vi "JudgeVoltage.vi"(9 "High_mV":i32, 10 "Low_mV":i32, 11 "Voltage_mV":i32) -> (2 "InputValid":bool, 3 "Result":u16)   [LabVIEW 2026]
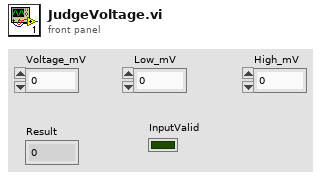
[diagram p1: front panel]
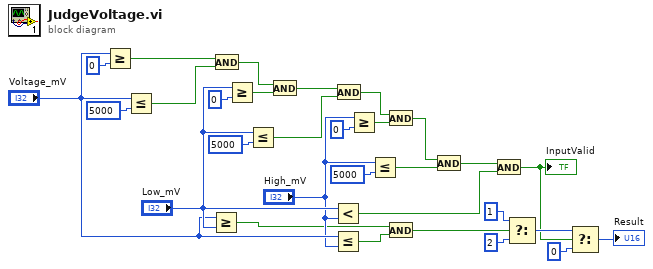
[diagram p0: block diagram]
diagram:
  n1 = Greater Or Equal?(x="Voltage_mV", y=0) -> (x >= y?=w24:bool)
  n2 = Less Or Equal?(x="Voltage_mV", y=5000) -> (x <= y?=w23:bool)
  n3 = Greater Or Equal?(x="Voltage_mV", y="Low_mV") -> (x >= y?=w9:bool)
  n4 = And(x=w24, y=w23) -> (x .and. y?=w22:bool)
  n5 = Greater Or Equal?(x="Low_mV", y=0) -> (x >= y?=w21:bool)
  n6 = Less Or Equal?(x="Low_mV", y=5000) -> (x <= y?=w19:bool)
  n7 = And(x=w22, y=w21) -> (x .and. y?=w20:bool)
  n8 = Less?(x="Low_mV", y="High_mV") -> (x < y?=w13:bool)
  n9 = Less Or Equal?(x="Voltage_mV", y="High_mV") -> (x <= y?=w8:bool)
  n10 = And(x=w20, y=w19) -> (x .and. y?=w18:bool)
  n11 = Greater Or Equal?(x="High_mV", y=0) -> (x >= y?=w17:bool)
  n12 = Less Or Equal?(x="High_mV", y=5000) -> (x <= y?=w15:bool)
  n13 = And(x=w18, y=w17) -> (x .and. y?=w16:bool)
  n14 = And(x=w9, y=w8) -> (x .and. y?=w7:bool)
  n15 = And(x=w16, y=w15) -> (x .and. y?=w14:bool)
  n16 = And(x=w14, y=w13) -> (x .and. y?=w3:bool)
  "InputValid" <- w3
  n17 = Select(t=u16 1, s=w7, f=u16 2) -> (s? t:f=w4:u16)
  n18 = Select(t=w4, s=w3, f=u16 0) -> (s? t:f=→"Result":u16)
